vi "Donnees fichier local.vi"() -> (0 "Données":string[](array[string]), 1 "données présentes":bool)   [LabVIEW 2022 SP3]
uses:
  Variables globales/Variable glob Keller.vi
  Variables globales/Variable glob Leybold.vi
  Variables globales/Variable glob Edwards.vi
  Variables globales/Variable glob Th.vi
  Variables globales/Variable glob Pt.vi
  Variables globales/Variables glob EUROTHERM.vi
  Variables globales/Variable globale compteurs.vi
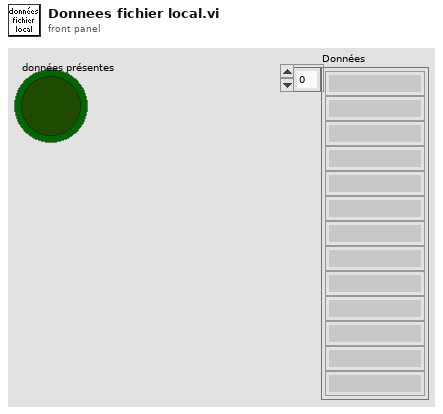
[diagram p1: front panel]
types:
  T1 = cluster{"Nom tache Pt":refnum<k21>, "Noms des Pt":string[], "Nb Pt":i16, "Selection Pt":bool[], "Nom Pt selectionnees":string[]}[]
  T2 = cluster{"Nom tache Th":refnum<k21>, "Noms des Th":string[], "Nb Th":i16, "Selection Th":bool[], "Nom Th selectionnes":string[]}[]
  T3 = cluster{"Nom tache compteurs":refnum<k21>, "Noms des compteurs":string[], "Selection":bool[], "Init compteurs":dbl[], "Noms compteurs selectionnes":string[]}
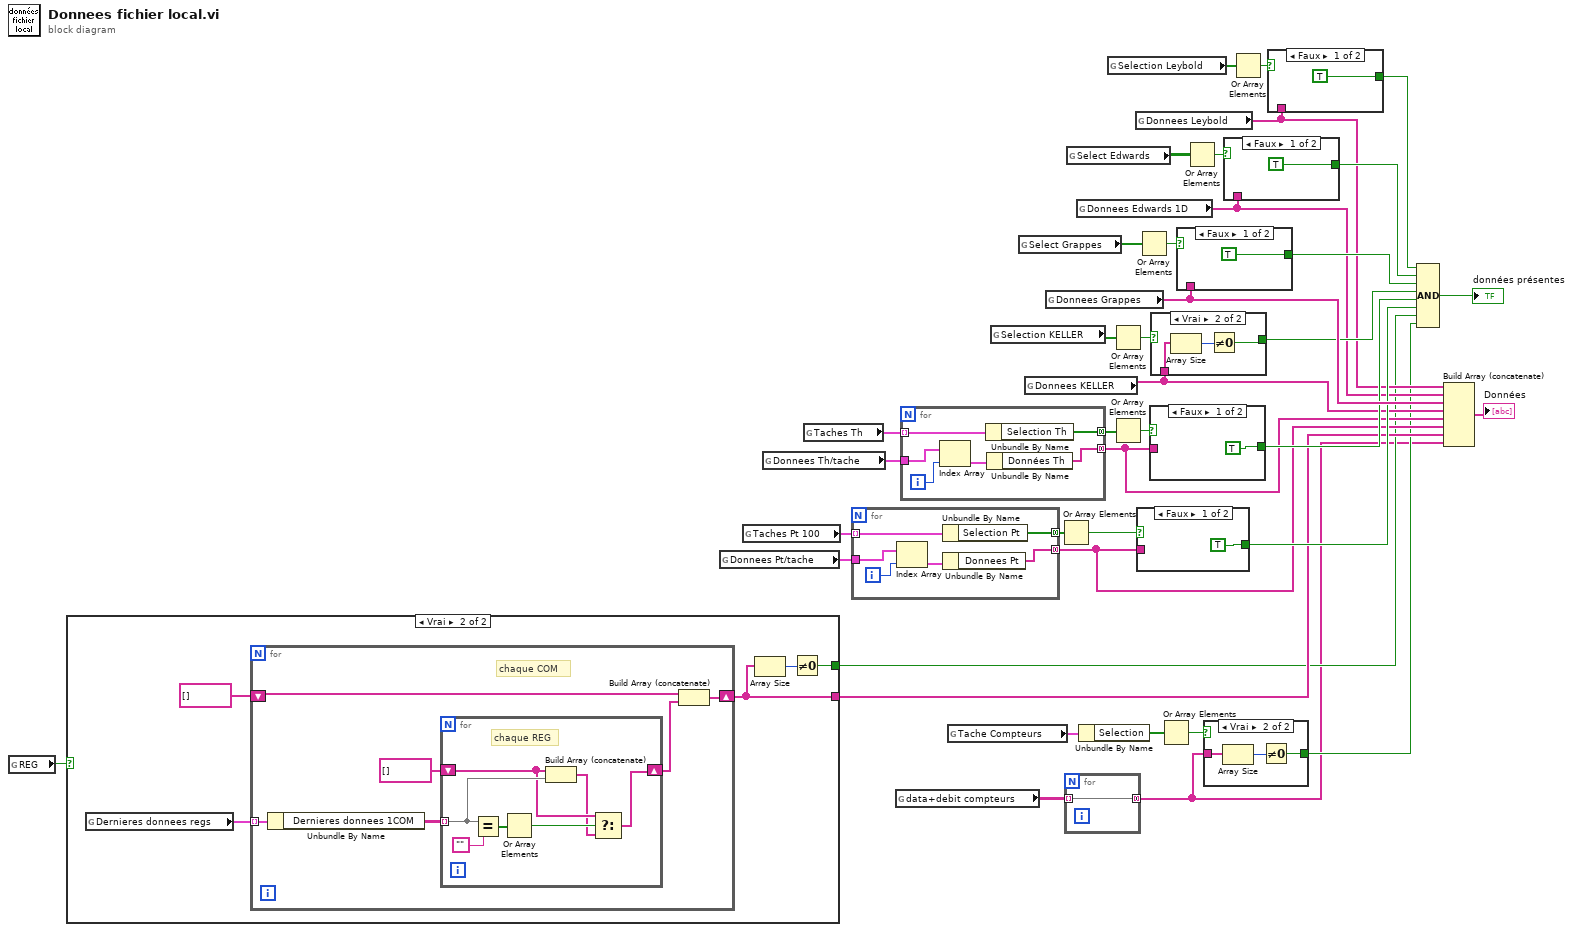
[diagram p0: block diagram]
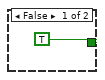
[diagram p2: hidden frame]
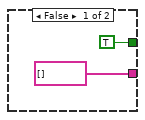
[diagram p3: hidden frame]
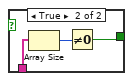
[diagram p4: hidden frame]
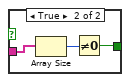
[diagram p5: hidden frame]
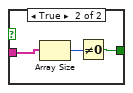
[diagram p6: hidden frame]
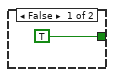
[diagram p7: hidden frame]
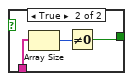
[diagram p8: hidden frame]
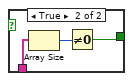
[diagram p9: hidden frame]
diagram:
  n1 = global read "Variables glob EUROTHERM.vi" "REG"() -> (w9:bool)
  n2 = case shown="Vrai" w9 {
    tunnel: [string[] [] w43] -> w8
    tunnel: [TRUE w42] -> w7
    frame False {
    }
    frame True {
      n3 = global read "Variables glob EUROTHERM.vi" "Dernieres donnees regs"() -> (w45:cluster{"Dernieres donnees 1COM":string[][]}[])
      n4 = for {
        tunnel: w45 -> [w48] mode=indexing
        shift-right: [w49] -> w43
        shift-left: string[] [] -> [w50]
        # "chaque COM"
        n5 = Unbundle By Name(w48) -> ("Dernieres donnees 1COM"=w47:string[][])
        n6 = for {
          tunnel: w47 -> [w59] mode=indexing
          shift-right: [w53] -> w51
          shift-left: string[] [] -> [w55]
          # "chaque REG"
          n7 = Equal?(x=w59, y="") -> (x = y?=w57:bool[])
          n8 = Or Array Elements(Boolean array=w57) -> (logical OR=w56:bool)
          n9 = Build Array (concatenate)(w55, w59) -> (w54:string[])
          n10 = Select(t=w55, s=w56, f=w54) -> (s? t:f=w53:string[])
        }
        n11 = Build Array (concatenate)(w50, w51) -> (w49:string[])
      }
      n12 = Array Size(array=w43) -> (size(s)=w44:i32)
      n13 = Not Equal To 0?(x=w44) -> (x != 0?=w42:bool)
    }
  }
  n14 = global read "Variable glob Pt.vi" "Donnees Pt/tache"() -> (w11:cluster{"Donnees Pt":string[]}[])
  n15 = global read "Variable glob Pt.vi" "Taches Pt 100"() -> (w17:T1)
  n16 = global read "Variable glob Th.vi" "Donnees Th/tache"() -> (w10:cluster{"Données Th":string[]}[])
  n17 = global read "Variable glob Th.vi" "Taches Th"() -> (w14:T2)
  n18 = for {
    tunnel: w17 -> [w65] mode=indexing
    tunnel: [w64] -> w16 mode=concatenating
    tunnel: [w63] -> w12 mode=concatenating
    tunnel: w11 -> [w62]
    i -> [w61]
    n19 = Index Array(array=w62, index=w61) -> (element=w60:cluster{"Donnees Pt":string[]})
    n20 = Unbundle By Name(w65) -> ("Selection Pt"=w64:bool[])
    n21 = Unbundle By Name(w60) -> ("Donnees Pt"=w63:string[])
  }
  n22 = global read "Variable globale compteurs.vi" "data+debit compteurs"() -> (w2:string[][])
  n23 = for {
    tunnel: w14 -> [w71] mode=indexing
    tunnel: [w70] -> w15 mode=concatenating
    tunnel: [w69] -> w13 mode=concatenating
    tunnel: w10 -> [w68]
    i -> [w67]
    n24 = Index Array(array=w68, index=w67) -> (element=w66:cluster{"Données Th":string[]})
    n25 = Unbundle By Name(w71) -> ("Selection Th"=w70:bool[])
    n26 = Unbundle By Name(w66) -> ("Données Th"=w69:string[])
  }
  n27 = global read "Variable globale compteurs.vi" "Tache Compteurs"() -> (w5:T3)
  n28 = global read "Variable glob Keller.vi" "Selection KELLER"() -> (w21:bool[])
  n29 = global read "Variable glob Edwards.vi" "Select Grappes"() -> (w37:bool[])
  n30 = global read "Variable glob Keller.vi" "Donnees KELLER"() -> (w28:string[])
  n31 = global read "Variable glob Edwards.vi" "Donnees Grappes"() -> (w38:string[])
  n32 = Or Array Elements(Boolean array=w16) -> (logical OR=w32:bool)
  n33 = for {
    tunnel: w2 -> [w72] mode=indexing
    tunnel: [w72] -> w1 mode=concatenating
  }
  n34 = global read "Variable glob Edwards.vi" "Select Edwards"() -> (w20:bool[][])
  n35 = global read "Variable glob Edwards.vi" "Donnees Edwards 1D"() -> (w25:string[])
  n36 = Unbundle By Name(w5) -> ("Selection"=w4:bool[])
  n37 = global read "Variable glob Leybold.vi" "Selection Leybold"() -> (w18:bool[])
  n38 = Or Array Elements(Boolean array=w21) -> (logical OR=w27:bool)
  n39 = Or Array Elements(Boolean array=w15) -> (logical OR=w30:bool)
  n40 = global read "Variable glob Leybold.vi" "Donnees Leybold"() -> (w19:string[])
  n41 = case shown="Faux" w32 {
    tunnel: [TRUE w75] -> w33
    tunnel: w12 -> [_ w74]
    frame False {
    }
    frame True {
      n42 = Array Size(array=w74) -> (size(s)=w76:i32)
      n43 = Not Equal To 0?(x=w76) -> (x != 0?=w75:bool)
    }
  }
  n44 = Or Array Elements(Boolean array=w37) -> (logical OR=w36:bool)
  n45 = case shown="Faux" w30 {
    tunnel: [TRUE w79] -> w31
    tunnel: w13 -> [_ w78]
    frame False {
    }
    frame True {
      n46 = Array Size(array=w78) -> (size(s)=w80:i32)
      n47 = Not Equal To 0?(x=w80) -> (x != 0?=w79:bool)
    }
  }
  n48 = case shown="Vrai" w27 {
    tunnel: w28 -> [_ w84]
    tunnel: [TRUE w82] -> w29
    frame False {
    }
    frame True {
      n49 = Array Size(array=w84) -> (size(s)=w83:i32)
      n50 = Not Equal To 0?(x=w83) -> (x != 0?=w82:bool)
    }
  }
  n51 = Or Array Elements(Boolean array=w4) -> (logical OR=w6:bool)
  n52 = case shown="Faux" w36 {
    tunnel: w38 -> [_ w88]
    tunnel: [TRUE w86] -> w39
    frame False {
    }
    frame True {
      n53 = Array Size(array=w88) -> (size(s)=w87:i32)
      n54 = Not Equal To 0?(x=w87) -> (x != 0?=w86:bool)
    }
  }
  n55 = Or Array Elements(Boolean array=w20) -> (logical OR=w24:bool)
  n56 = case shown="Vrai" w6 {
    tunnel: w1 -> [_ w92]
    tunnel: [TRUE w90] -> w3
    frame False {
    }
    frame True {
      n57 = Array Size(array=w92) -> (size(s)=w91:i32)
      n58 = Not Equal To 0?(x=w91) -> (x != 0?=w90:bool)
    }
  }
  n59 = case shown="Faux" w24 {
    tunnel: w25 -> [_ w96]
    tunnel: [TRUE w94] -> w26
    frame False {
    }
    frame True {
      n60 = Array Size(array=w96) -> (size(s)=w95:i32)
      n61 = Not Equal To 0?(x=w95) -> (x != 0?=w94:bool)
    }
  }
  n62 = Or Array Elements(Boolean array=w18) -> (logical OR=w22:bool)
  n63 = case shown="Faux" w22 {
    tunnel: w19 -> [_ w100]
    tunnel: [TRUE w98] -> w23
    frame False {
    }
    frame True {
      n64 = Array Size(array=w100) -> (size(s)=w99:i32)
      n65 = Not Equal To 0?(x=w99) -> (x != 0?=w98:bool)
    }
  }
  n66 = Compound Arithmetic op=AND(w23, w26, w39, w29, w31, w33, w7, w3) -> (→"données présentes":bool)
  n67 = Build Array (concatenate)(w19, w25, w38, w28, w13, w12, w8, w1) -> (→"Données":string[])
